vi "Get SubVI Terminal (by Name).vi"(8 "error in (no error)":errorcluster, 10 "Terminal name":string, 11 "SubVI in":refnum<vi>) -> (0 "error out":errorcluster, 1 "Found?":bool, 2 "SubVI Term ref":refnum<vi>, 3 "SubVI out":refnum<vi>)   [LabVIEW 2019, in "gRPC Template Creation Utility.lvlib"]
uses:
  gRPC Template Creation Utility.lvlib
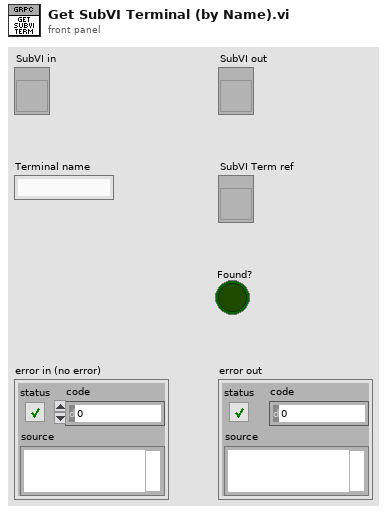
[diagram p1: front panel]
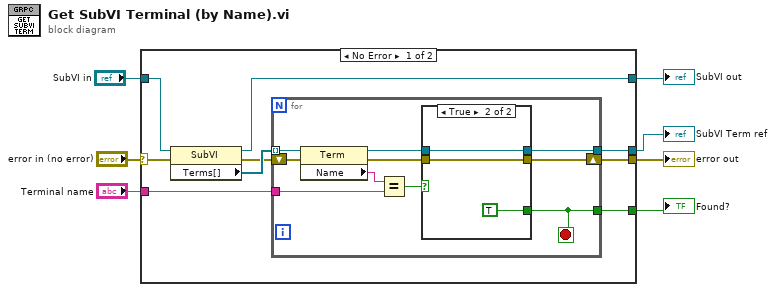
[diagram p0: block diagram]
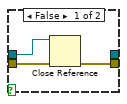
[diagram p2: hidden frame]
diagram:
  n1 = case shown="No Error" "error in (no error)" {
    selector: "error in (no error)" -> [w10 w34]
    tunnel: "Terminal name" -> [w16 _]
    tunnel: [w8 w34] -> w6
    tunnel: "SubVI in" -> [w14 w33]
    tunnel: [w11 w33] -> w2
    tunnel: [w15 _] -> w4
    tunnel: [w12 _] -> w1
    frame No Error {
      n2 = property class="SubVI"(reference=w14, error in=w10) -> (reference out=w11:refnum<vi>, error out=w9:errorcluster, "Terms[]"=w13:refnum<vi>[])
      n3 = for {
        tunnel: w16 -> [w26]
        tunnel: [w24] -> w15
        tunnel: w13 -> [w23] mode=indexing
        tunnel: [w21] -> w12
        shift-right: [w17] -> w8
        shift-left: w9 -> [w20]
        stop <- w24 stop-if-true
        n4 = property class="Term"(reference=w23, error in=w20) -> (reference out=w22:refnum<vi>, error out=w18:errorcluster, "Name"=w19:string)
        n5 = Equal?(x=w19, y=w26) -> (x = y?=w25:bool)
        n6 = case shown="True" w25 {
          tunnel: [_ TRUE] -> w24
          tunnel: w22 -> [w29 w31]
          tunnel: [_ w31] -> w21
          tunnel: w18 -> [w28 w30]
          tunnel: [w27 w30] -> w17
          frame False {
            n7 = Close Reference(reference=w29, error in (no error)=w28) -> (error out=w27:errorcluster)
          }
          frame True {
          }
        }
      }
    }
    frame Error {
    }
  }
  "error out" <- w6
  "Found?" <- w4
  "SubVI out" <- w2
  "SubVI Term ref" <- w1
